vi "ParseDependencyList.vi"(8 "Error In":errorcluster, 11 "Depends":string) -> (0 "Error Out":errorcluster, 3 "DependencyRelationships":T1[](array[typedef]))   [LabVIEW 2019, in "CEPM.lvlib"]
uses:
  CEPM.lvlib
  Typedefs/DependencyRelationship.ctl
  <vilib>/regexp/Match Regular Expression.xnode
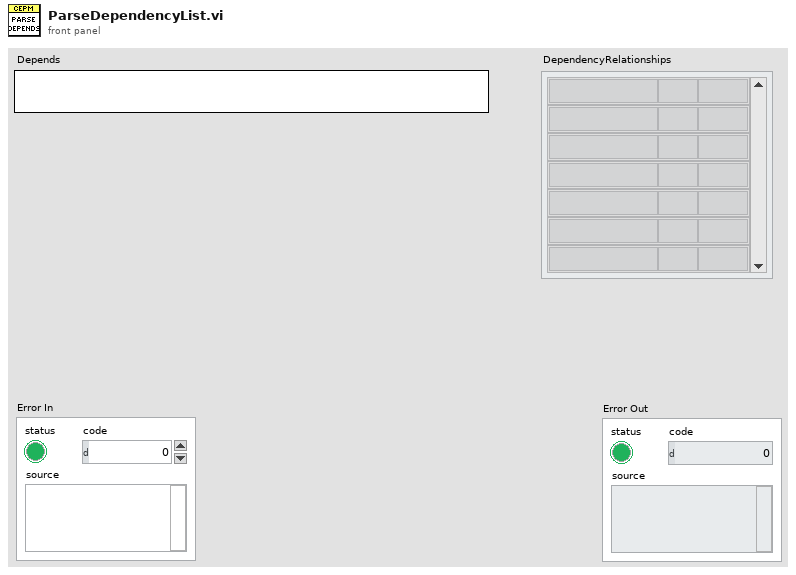
[diagram p1: front panel]
types:
  T1 = typedef "DependencyRelationship.ctl" = cluster{"Package":string, "Relation":string, "Version":string}
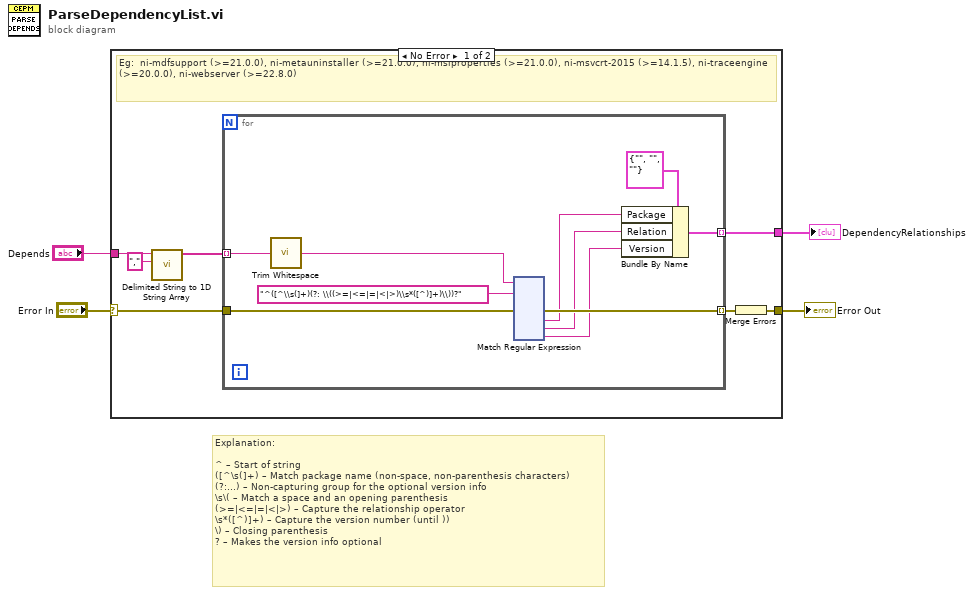
[diagram p0: block diagram]
diagram:
  # "Explanation:\n\n^ – Start of string\n([^\\s(]+) – Match package name (non-space, non-parenthesis characters)\n(?:...) – Non-capturing group for the optional version info\n\\s\\( – Match a space and an opening parenthesis\n(>=|<=|=|<|>) – Capture the relationship operator\n\\s*([^)]+) – Capture the version number (until ))\n\\) – Closing parenthesis\n? – Makes the version info optional"
  n1 = case shown="No Error" "Error In" {
    selector: "Error In" -> [w7 w140]
    tunnel: [w5 w140] -> w3
    tunnel: "Depends" -> [w11 _]
    tunnel: [w8 _] -> w1
    frame No Error {
      # "Eg:  ni-mdfsupport (>=21.0.0), ni-metauninstaller (>=21.0.0), ni-msiproperties (>=21.0.0), ni-msvcrt-2015 (>=14.1.5), ni-traceengine (>=20.0.0), ni-webserver (>=22.8.0)"
      n2 = call <vilib>:"Delimited String to 1D String Array.vi"("delimiter"=",", "delimited string"=w11) -> ("string array"=w9:string[])  [unwired: 9 in]
      n3 = for {
        tunnel: w9 -> [w16] mode=indexing
        tunnel: [w20] -> w8 mode=indexing
        tunnel: w7 -> [w18]
        tunnel: [w17] -> w6 mode=indexing
        n4 = call <vilib>:"Trim Whitespace.vi"("string"=w16) -> ("trimmed string"=w12:string)  [unwired: 1 in]
        n5 = xnode "Match Regular Expression"("input string"=w12, "regular expression"="^([^\\s(]+)(?: \\((>=|<=|=|<|>)\\s*([^)]+)\\))?", "error in"=w18) -> ("error out"=w17:errorcluster, "submatch 1"=w15:string, "submatch 2"=w14:string, "submatch 3"=w13:string)  [unwired: 3 in, 4 out]
        n6 = Bundle By Name(cluster=T1 {"Package"="", "Relation"="", "Version"=""} ("DependencyRelationship"), "Package"=w15, "Relation"=w14, "Version"=w13) -> (w20:T1)
      }
      n7 = Merge Errors(w6) -> (w5:errorcluster)
    }
    frame Error {
    }
  }
  "Error Out" <- w3
  "DependencyRelationships" <- w1
